vi "Simulation ThermistorWithLED (1).vi"() -> ()   [LabVIEW 2026]
panel:
  out "Status":string
  in  "Cool Thermistor":bool
  in  "Heat Thermistor":bool
  out "Thermistor Color State":string="Neutral"
  in  "Min Temp (F)":dbl
  in  "Max Temp (F)":dbl
  out "Temp (C)":dbl
  out "Temp (F)":dbl
  out "Overtemp Warning":bool
  out "Undertemp Warning":bool
  in  "Stop":bool
  out "Temperature (F)":dbl(graph)=24.253996937637567
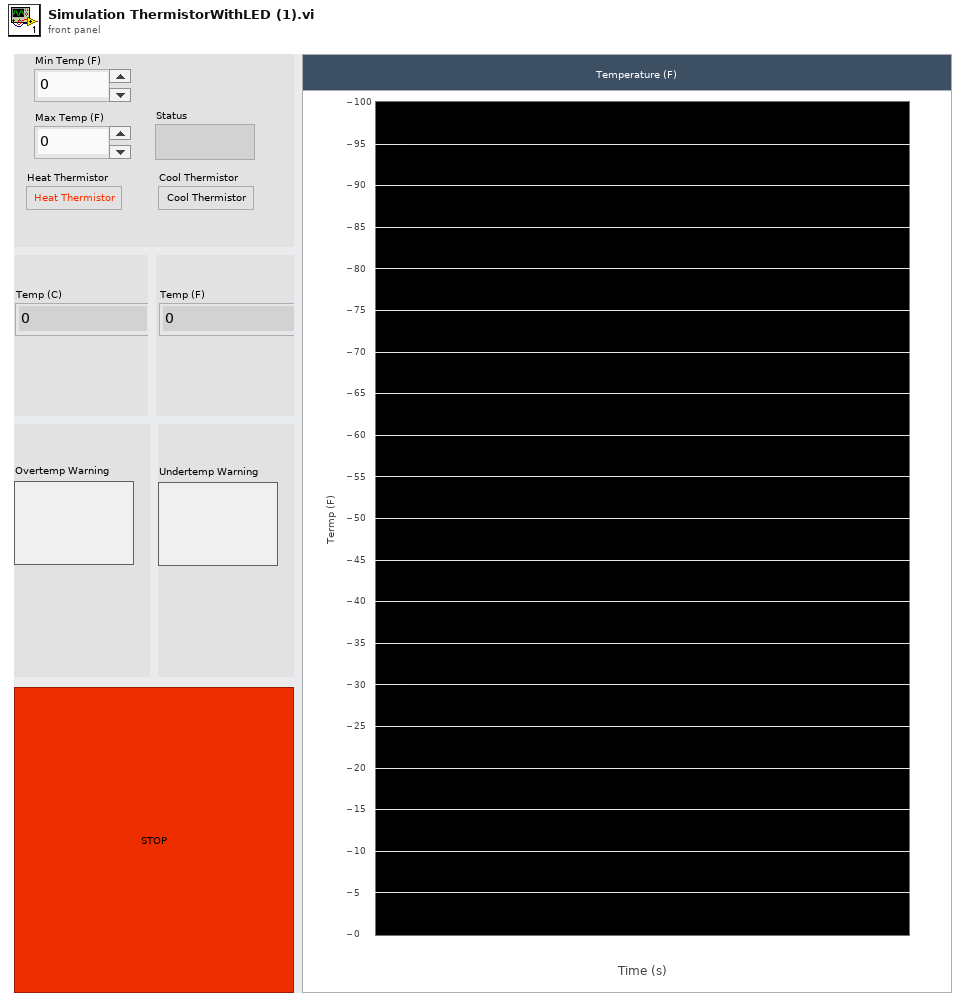
[diagram p1: front panel]
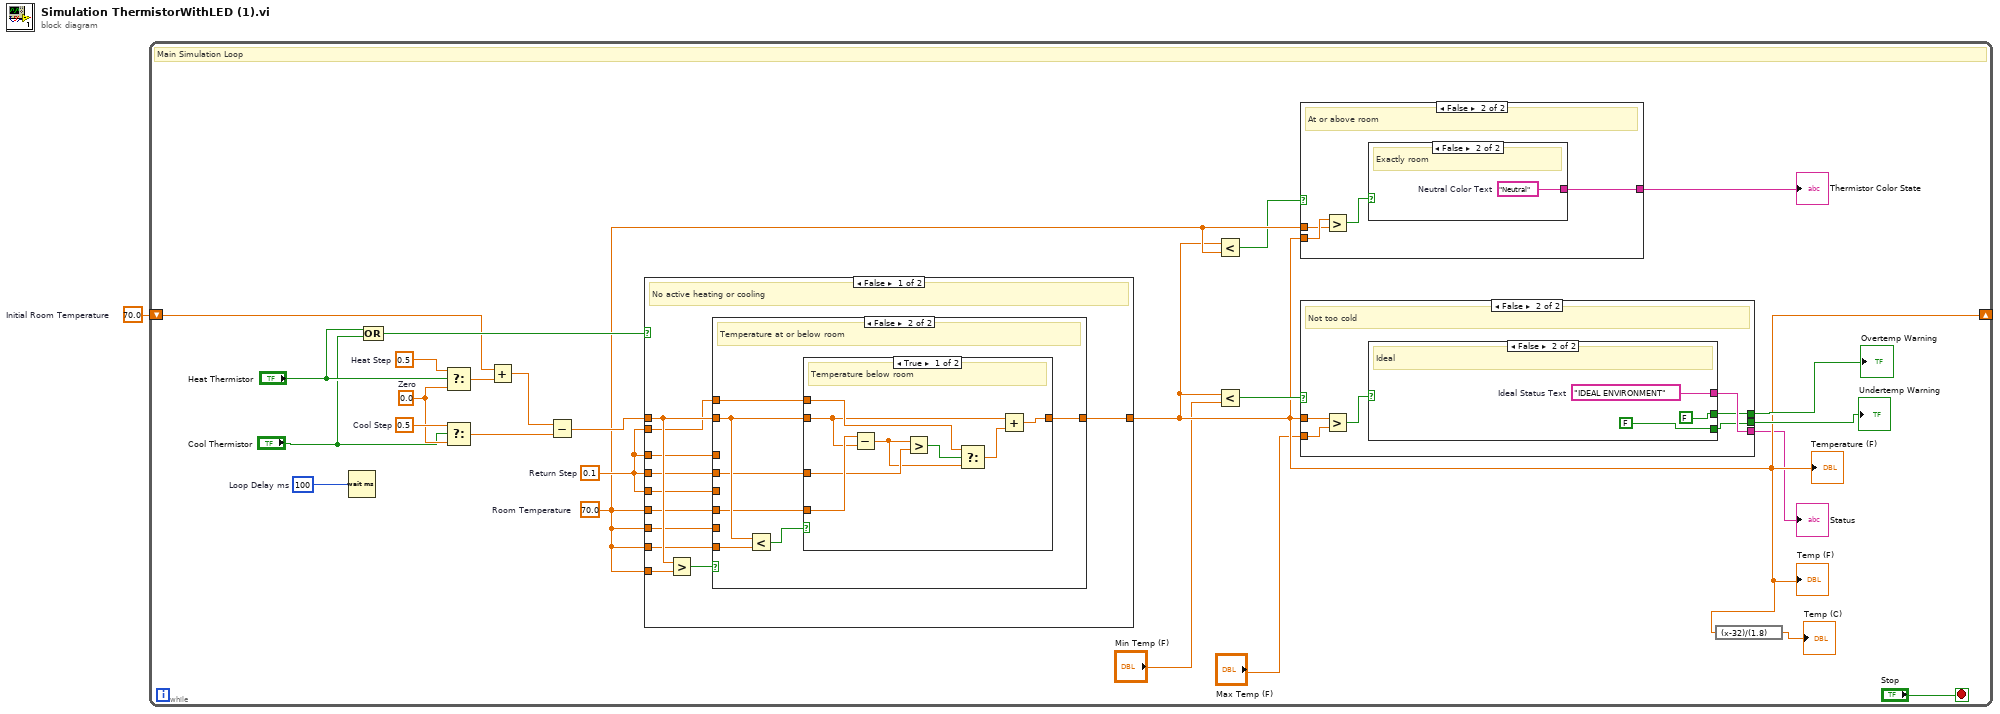
[diagram p0: block diagram]
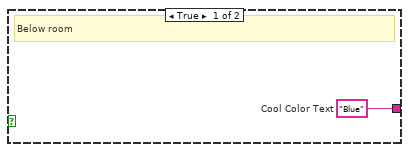
[diagram p2: hidden frame]
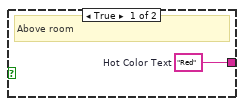
[diagram p3: hidden frame]
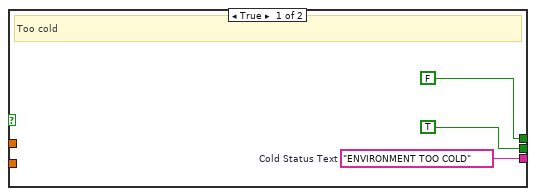
[diagram p4: hidden frame]
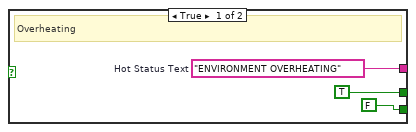
[diagram p5: hidden frame]
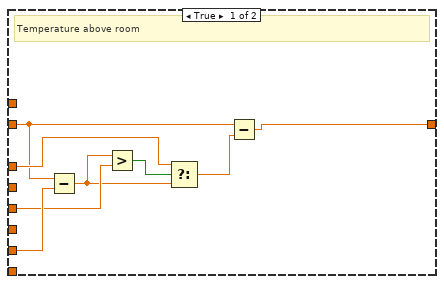
[diagram p6: hidden frame]
diagram:
  w1 = 70.0  # Initial Room Temperature
  n1 = while {
    shift-right: [w6] -> _
    shift-left: w1 -> [w12]
    stop <- "Stop" stop-if-true
    w13 = u32 100  # Loop Delay ms
    w19 = 0.1  # Return Step
    w16 = 70.0  # Room Temperature
    w24 = 0.0  # Zero
    w25 = 0.5  # Cool Step
    w26 = 0.5  # Heat Step
    # "Main Simulation Loop"
    n2 = Wait (ms)(milliseconds to wait=w13) -> ()  [unwired: 1 out]
    n3 = Compound Arithmetic op=OR("Heat Thermistor", "Cool Thermistor") -> (w18:bool)
    n4 = Select(t=w26, s="Heat Thermistor", f=w24) -> (s? t:f=w23:dbl)
    n5 = Select(t=w25, s="Cool Thermistor", f=w24) -> (s? t:f=w21:dbl)
    n6 = Add(x=w12, y=w23) -> (x+y=w22:dbl)
    n7 = Subtract(x=w22, y=w21) -> (x-y=w20:dbl)
    n8 = case shown="False" w18 {
      tunnel: w20 -> [w58 w84]
      tunnel: w16 -> [w59 _]
      tunnel: w16 -> [w57 _]
      tunnel: w19 -> [w56 _]
      tunnel: w19 -> [w55 _]
      tunnel: w16 -> [w54 _]
      tunnel: w16 -> [w53 _]
      tunnel: w19 -> [w52 _]
      tunnel: w19 -> [w51 _]
      tunnel: [w49 w84] -> w6
      frame False {
        # "No active heating or cooling"
        n9 = Greater?(x=w58, y=w59) -> (0:w50:bool)
        n10 = case shown="False" w50 {
          tunnel: w58 -> [w62 w73]
          tunnel: w57 -> [w67 _]
          tunnel: w56 -> [w66 _]
          tunnel: w55 -> [w65 _]
          tunnel: [w60 w68] -> w49
          tunnel: w54 -> [_ w74]
          tunnel: w53 -> [_ w72]
          tunnel: w52 -> [_ w71]
          tunnel: w51 -> [_ w70]
          frame True {
            # "Temperature above room"
            n11 = Subtract(x=w62, y=w67) -> (x-y=w63:dbl)
            n12 = Greater?(x=w63, y=w66) -> (0:w64:bool)
            n13 = Select(t=w65, s=w64, f=w63) -> (s? t:f=w61:dbl)
            n14 = Subtract(x=w62, y=w61) -> (x-y=w60:dbl)
          }
          frame False {
            # "Temperature at or below room"
            n15 = Less?(x=w73, y=w74) -> (x < y?=w69:bool)
            n16 = case shown="True" w69 {
              tunnel: w73 -> [w77 w83]
              tunnel: w72 -> [w82 _]
              tunnel: w71 -> [w81 _]
              tunnel: w70 -> [w80 _]
              tunnel: [w75 w83] -> w68
              frame True {
                # "Temperature below room"
                n17 = Subtract(x=w82, y=w77) -> (x-y=w78:dbl)
                n18 = Greater?(x=w78, y=w81) -> (0:w79:bool)
                n19 = Select(t=w80, s=w79, f=w78) -> (s? t:f=w76:dbl)
                n20 = Add(x=w77, y=w76) -> (x+y=w75:dbl)
              }
              frame False {
                # "Temperature exactly room"
              }
            }
          }
        }
      }
      frame True {
        # "Heating or cooling active"
      }
    }
    "Temperature (F)" <- w6
    "Temp (F)" <- w6
    n21 = Less?(x=w6, y=w16) -> (x < y?=w14:bool)
    n22 = Less?(x=w6, y="Min Temp (F)") -> (x < y?=w17:bool)
    n23 = case shown="False" w14 {
      tunnel: [w27 w28] -> w15
      tunnel: w6 -> [_ w31]
      tunnel: w16 -> [_ w30]
      frame True {
        w27 = "Blue"  # Cool Color Text
        # "Below room"
      }
      frame False {
        # "At or above room"
        n24 = Greater?(x=w31, y=w30) -> (0:w29:bool)
        n25 = case shown="False" w29 {
          tunnel: [w32 w33] -> w28
          frame True {
            w32 = "Red"  # Hot Color Text
            # "Above room"
          }
          frame False {
            w33 = "Neutral"  # Neutral Color Text
            # "Exactly room"
          }
        }
      }
    }
    "Thermistor Color State" <- w15
    n26 = case shown="False" w17 {
      tunnel: [w36 w39] -> w2
      tunnel: w6 -> [_ w42]
      tunnel: "Max Temp (F)" -> [_ w41]
      tunnel: [FALSE ("Overtemp Warning") w38] -> w8
      tunnel: [TRUE ("Undertemp Warning") w37] -> w7
      frame True {
        w36 = "ENVIRONMENT TOO COLD"  # Cold Status Text
        # "Too cold"
      }
      frame False {
        # "Not too cold"
        n27 = Greater?(x=w42, y=w41) -> (0:w40:bool)
        n28 = case shown="False" w40 {
          tunnel: [w45 w48] -> w39
          tunnel: [TRUE ("Overtemp Warning") FALSE ("Overtemp Warning")] -> w38
          tunnel: [FALSE ("Undertemp Warning") FALSE ("Undertemp Warning")] -> w37
          frame True {
            w45 = "ENVIRONMENT OVERHEATING"  # Hot Status Text
            # "Overheating"
          }
          frame False {
            w48 = "IDEAL ENVIRONMENT"  # Ideal Status Text
            # "Ideal"
          }
        }
      }
    }
    "Overtemp Warning" <- w8
    "Undertemp Warning" <- w7
    "Status" <- w2
    n29 = expression code="(x-32)/(1.8)"(w6) -> (→"Temp (C)":dbl)
  }
